vi "Get Resource.vi"(8 "error in (no error)":errorcluster, 11 "Device in":refnum<class "Device.lvclass">) -> (0 "error out":errorcluster, 2 "Resource":string, 3 "Device out":refnum<class "Device.lvclass">)   [LabVIEW 2020, in "HAL.lvlib" / "Device.lvclass"]
doc: "All concrete device classes need to override this VI to provide a string representation of the device's connection means or address. This is used to differentiate multiple different devices of the same model if configured in the editor. IE two of the same model power supplies but one connects via COM4 and the second connects via COM5. The concrete device still needs to store configuration value(s) for the resource on its own, for instance by setting Port = COM4 with the Set Config Value VI, as this is only provided as a means for displaying readable values in the configuration editor."
uses:
  Device.lvclass
  <vilib>/Utility/error.llb/Error Cluster From Error Code.vi
  <vilib>/ErrorRing/Error Ring.xnode
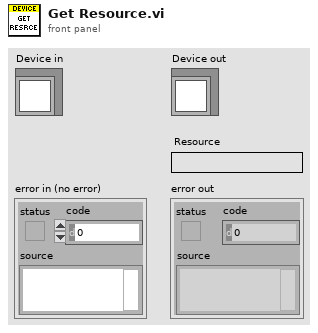
[diagram p1: front panel]
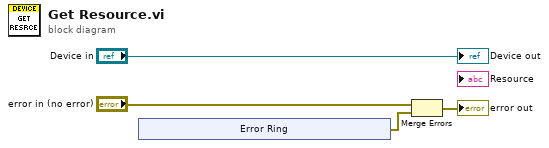
[diagram p0: block diagram]
diagram:
  n1 = xnode "Error Ring"() -> ("error out"=w1:errorcluster)
  n2 = Merge Errors("error in (no error)", w1) -> (→"error out":errorcluster)
  "Device out" <- "Device in"
